vi "SeqEditor_StepMLST-ReNameBoxValueChange.vi"(8 "error in (no error)":errorcluster, 11 "NLTest in":refnum<class "NLTest.lvclass">) -> (0 "error out":errorcluster, 3 "NLTest out":refnum<class "NLTest.lvclass">)   [LabVIEW 2017, in "NLTest.lvclass"]
uses:
  NLTest.lvclass
  VISTEP.ctl
  VISTEP_class_INOUTPUT.ctl
  VISTEP_class_INOUTPUT_TYPE.ctl
  NLTest.lvclass/NLTest.ctl
  SeqEditor_Global.vi
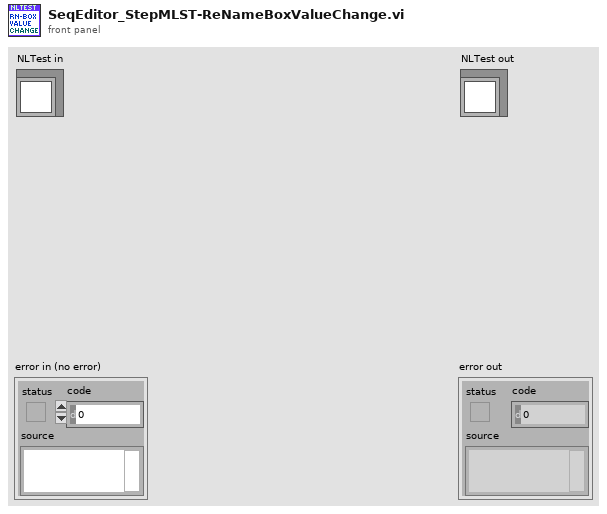
[diagram p1: front panel]
types:
  T1 = typedef "NLTest.lvclass/VISTEP.ctl" = cluster{"My":cluster{"VIpath":T2, "VIname":T2, "Loop":T2, "Skip":T2, "FailStop":T2, "StepClass":T2, "StringTest-Source":T2, "StringTest-Lim":T2, "BoolTest-Source":T2, "BoolTest-Lim":T2, "NumberTest-OP":T2, "NumberTest-Source":T2, "NumberTest-LimA":T2, "NumberTest-LimB":T2}, "INPUT":T2[], "OUTPUT":T2[]}
  T2 = typedef "NLTest.lvclass/VISTEP_class_INOUTPUT.ctl" = cluster{"ITEM":string, "DATA":string, "TYPE":T3, "TYPEDATA":string, "SV":bool, "clusterchain":refnum<vi>[]}
  T3 = typedef "NLTest.lvclass/VISTEP_class_INOUTPUT_TYPE.ctl" = enum16{"Number", "String", "Bool", "Enum", "Path", "VISA", "NA"}
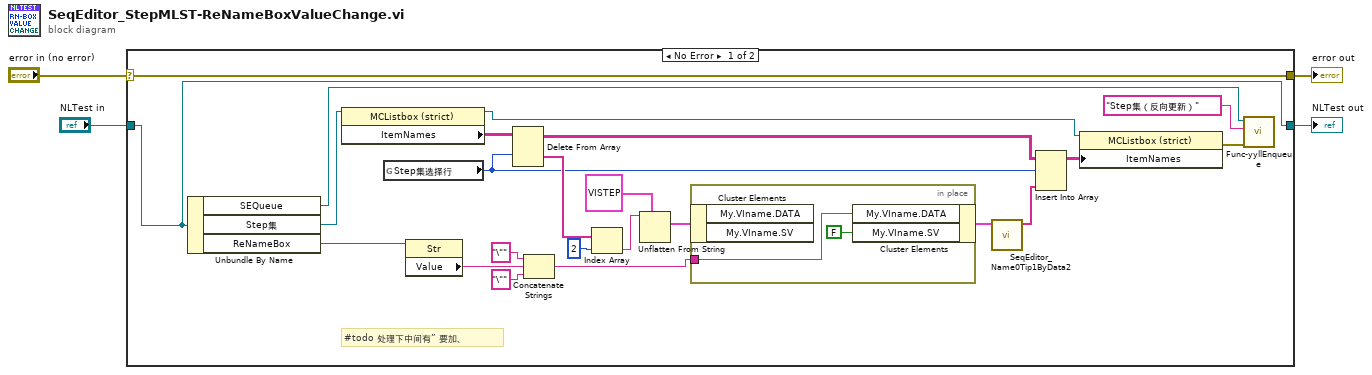
[diagram p0: block diagram]
diagram:
  n1 = case shown="No Error" "error in (no error)" {
    selector: "error in (no error)" -> [w27 w31]
    tunnel: [w27 w31] -> w3
    tunnel: [w26 w30] -> w1
    tunnel: "NLTest in" -> [w26 w30]
    frame No Error {
      # "#todo 处理下中间有” 要加、"
      n2 = Unbundle By Name(w26) -> ("SEQueue"=w24:refnum<queue>, "Step集"=w23:refnum<vi>, "ReNameBox"=w20:refnum<vi>)
      n3 = property class="MCListbox (strict)"(reference=w23) -> (reference out=w22:refnum<vi>, "ItemNames"=w13:string[][])  [unwired: 1 in, 1 out]
      n4 = global read "SeqEditor_Global.vi" "Step集选择行"() -> (w7:i32)
      n5 = property class="Str"(reference=w20) -> ("Value"=w19:string)  [unwired: 1 in, 2 out]
      n6 = Delete From Array(array=w13, index (row)=w7) -> (deleted portion=w12:string[], array with subset deleted=w8:string[][])  [unwired: 2 in]
      n7 = Concatenate Strings("\"" ("string"), w19, "\"" ("string")) -> (w16:string)
      n8 = Index Array(array=w12, index=2 ("disabled index (col)")) -> (element=w10:string)
      n9 = Unflatten From String(type=T1 {"My"={"VIpath"={"ITEM"="VI路径", "DATA"="\"\"", "TYPE"=enum."Path", "TYPEDATA"="", "SV"=FALSE, "clusterchain"=[]}, "VIname"={"ITEM"="步骤名称", "DATA"="\"\"", "TYPE"=enum."String", "TYPEDATA"="", "SV"=FALSE, "clusterchain"=[]}, "Loop"={"ITEM"="重测次数", "DATA"="1", "TYPE"=enum."Number", "TYPEDATA"="", "SV"=FALSE, "clusterchain"=[]}, "Skip"={"ITEM"="跳过步骤", "DATA"="FALSE", "TYPE"=enum."Bool", "TYPEDATA"="", "SV"=FALSE, "clusterchain"=[]}, "FailStop"={"ITEM"="失败停止", "DATA"="FALSE", "TYPE"=enum."Bool", "TYPEDATA"="", "SV"=FALSE, "clusterchain"=[]}, "StepClass"={"ITEM"="步骤类型", "DATA"="NotaTEST", "TYPE"=enum."Enum", "TYPEDATA"="", "SV"=FALSE, "clusterchain"=[]}, "StringTest-Source"={"ITEM"="字符串测试值", "DATA"="\"\"", "TYPE"=enum."String", "TYPEDATA"="", "SV"=FALSE, "clusterchain"=[]}, "StringTest-Lim"={"ITEM"="字符串测试门限", "DATA"="\"\"", "TYPE"=enum."String", "TYPEDATA"="", "SV"=FALSE, "clusterchain"=[]}, "BoolTest-Source"={"ITEM"="布尔测试值", "DATA"="TRUE", "TYPE"=enum."Bool", "TYPEDATA"="", "SV"=FALSE, "clusterchain"=[]}, "BoolTest-Lim"={"ITEM"="布尔测试门限", "DATA"="TRUE", "TYPE"=enum."Bool", "TYPEDATA"="", "SV"=FALSE, "clusterchain"=[]}, "NumberTest-OP"={"ITEM"="数值测试OP", "DATA"="NotaTEST", "TYPE"=enum."Enum", "TYPEDATA"="", "SV"=FALSE, "clusterchain"=[]}, "NumberTest-Source"={"ITEM"="数值测试值", "DATA"="0", "TYPE"=enum."Number", "TYPEDATA"="", "SV"=FALSE, "clusterchain"=[]}, "NumberTest-LimA"={"ITEM"="数值测试门限A", "DATA"="0", "TYPE"=enum."Number", "TYPEDATA"="", "SV"=FALSE, "clusterchain"=[]}, "NumberTest-LimB"={"ITEM"="数值测试门限B", "DATA"="0", "TYPE"=enum."Number", "TYPEDATA"="", "SV"=FALSE, "clusterchain"=[]}}, "INPUT"=[], "OUTPUT"=[]} ("步骤结构"), binary string=w10) -> (value=w14:T1)  [unwired: 3 in, 2 out]
      n10 = in-place {
        in-place-border: w16 -> [w29]
        n11 = in-place-cluster #1(w14) -> ()  [unwired: 2 out]
        n12 = in-place-cluster #1("My.VIname.DATA"=w29, "My.VIname.SV"=FALSE) -> (w9:T1)
      }
      n13 = call "SeqEditor_Name0Tip1ByData2.vi"("output cluster"=w9) -> ("Array"=w6:string[])  [unwired: 10 in]
      n14 = Insert Into Array(array=w8, index (row)=w7, new element=w6) -> (w5:string[][])  [unwired: 1 in]
      n15 = property class="MCListbox (strict)"(reference=w22, "ItemNames"=w5) -> (error out=w21:errorcluster)  [unwired: 1 in, 1 out]
      n16 = call "Func-yyllEnqueue.vi"("error in (no error)"=w21, "cmd"="Step集（反向更新）", "queue in"=w24) -> ()  [unwired: 6 in, 3 out]
    }
    frame Error {
    }
  }
  "error out" <- w3
  "NLTest out" <- w1
